vi "PPMU Level Settings Extract.vi"(9 "Pin Name":string, 11 ".digilevel File Path":path) -> (0 "IRange":dbl, 1 "Vcl":dbl, 2 "Vch":dbl, 3 "If":dbl, 5 "Vf":dbl)   [LabVIEW 2025, in "Digital Pattern Sequencer.lvclass"]
uses:
  Digital Pattern Sequencer.lvclass
  Digital Pattern Sequencer.lvclass/Digital Pattern Sequencer.ctl
  <vilib>/xml/NI_XML.lvlib
  <resource>/objmgr/DOMUserDefRef.rc
  <vilib>/xml/Load XML String.vi
  <vilib>/xml/XPath/Get All Matched Nodes (String).vi
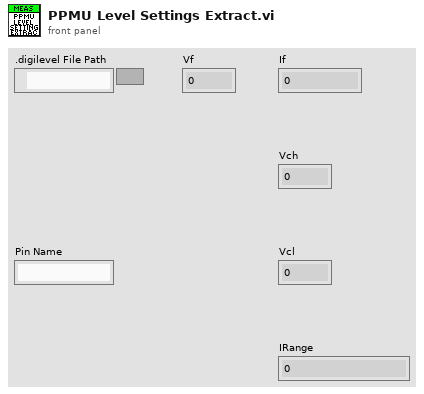
[diagram p1: front panel]
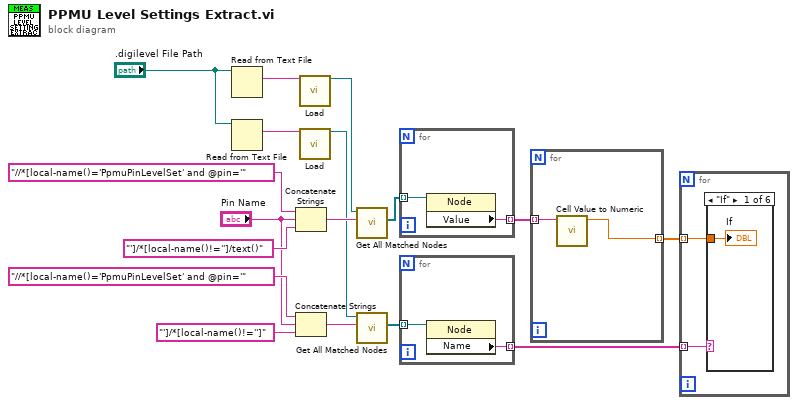
[diagram p0: block diagram]
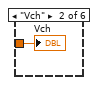
[diagram p2: hidden frame]
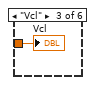
[diagram p3: hidden frame]
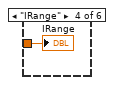
[diagram p4: hidden frame]
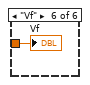
[diagram p6: hidden frame]
diagram:
  n1 = Read from Text File(file (use dialog)=".digilevel File Path") -> (text=w15:string)  [unwired: 3 in, 3 out]
  n2 = Read from Text File(file (use dialog)=".digilevel File Path") -> (text=w9:string)  [unwired: 3 in, 3 out]
  n3 = Concatenate Strings("//*[local-name()='PpmuPinLevelSet' and @pin='" ("string"), "Pin Name", "']/*[local-name()!='']/text()" ("string")) -> (w14:string)
  n4 = Concatenate Strings("//*[local-name()='PpmuPinLevelSet' and @pin='" ("string"), "Pin Name", "']/*[local-name()!='']" ("string")) -> (w4:string)
  n5 = call-poly <vilib>:"Load.vi"("XML string"=w15) -> ("DOM document out"=w16:refnum<k20>)  [unwired: 12 in, 2 out]
  n6 = call-poly <vilib>:"Load.vi"("XML string"=w9) -> ("DOM document out"=w10:refnum<k20>)  [unwired: 12 in, 2 out]
  n7 = call-poly <vilib>:"Get All Matched Nodes.vi"("XPath expression"=w14, "node in"=w16) -> ("node result array"=w17:refnum<k20>[])  [unwired: 7 in, 2 out]
  n8 = call-poly <vilib>:"Get All Matched Nodes.vi"("XPath expression"=w4, "node in"=w10) -> ("node result array"=w8:refnum<k20>[])  [unwired: 7 in, 2 out]
  n9 = for {
    tunnel: w17 -> [w19] mode=indexing
    tunnel: [w18] -> w11 mode=indexing
    n10 = property class="Node"(reference=w19) -> ("Value"=w18:string)  [unwired: 1 in, 2 out]
  }
  n11 = for {
    tunnel: w8 -> [w21] mode=indexing
    tunnel: [w20] -> w7 mode=indexing
    n12 = property class="Node"(reference=w21) -> ("Name"=w20:string)  [unwired: 1 in, 2 out]
  }
  n13 = for {
    tunnel: w11 -> [w23] mode=indexing
    tunnel: [w22] -> w6 mode=indexing
    n14 = call "Cell Value to Numeric.vi"("Cell Value"=w23) -> ("Numeric"=w22:dbl)  [unwired: 9 in, 1 out]
  }
  n15 = for {
    tunnel: w7 -> [w25] mode=indexing
    tunnel: w6 -> [w24] mode=indexing
    n16 = case shown="\"If\"" w25 {
      tunnel: w24 -> [w26 w27 w28 w29 _ w30]
      frame "If" {
        "If" <- w26
      }
      frame "Vch" {
        "Vch" <- w27
      }
      frame "Vcl" {
        "Vcl" <- w28
      }
      frame "IRange" {
        "IRange" <- w29
      }
      frame Default {
      }
      frame "Vf" {
        "Vf" <- w30
      }
    }
  }
